vi "POST-Call.vi"(8 "error in (no error)":errorcluster, 9 "FunctionCall":T1, 10 "ApiKey":string, 11 "BaseUrl":string) -> (0 "error out":errorcluster, 3 "ToolReturn":cluster{"id":string, "result":variant})   [LabVIEW 2017]
uses:
  <vilib>/httpClient/POSTBuffer.vi
  <vilib>/httpClient/LabVIEWHTTPClient.lvlib
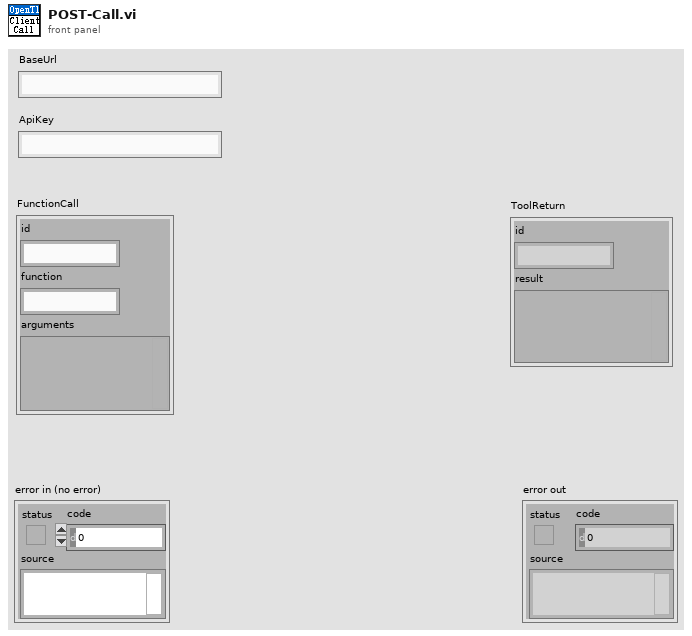
[diagram p1: front panel]
types:
  T1 = cluster{"id":string, "function":string, "arguments":variant}
  T2 = cluster{"jsonrpc":string, "id":string, "method":string, "params":variant}
  T3 = typedef "LabVIEWHTTPClient.lvlib/ClientHandle.ctl" = refnum<k1>
  T4 = cluster{"jsonrpc":string, "result":variant, "id":string, "JsonRPCHttpResponseBodyError":cluster{"code":i32, "message":string}}
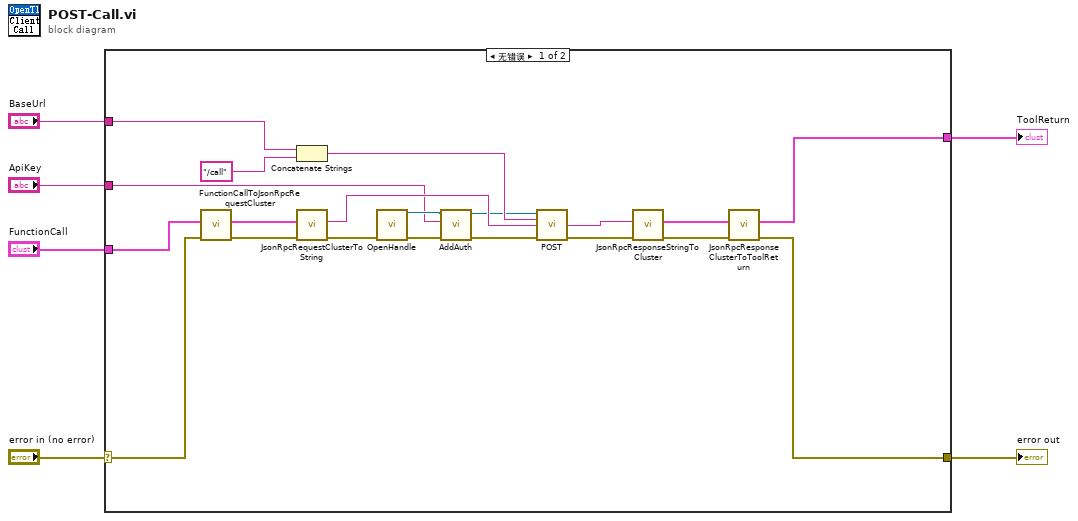
[diagram p0: block diagram]
diagram:
  n1 = case shown="无错误" "error in (no error)" {
    selector: "error in (no error)" -> [w16 w27]
    tunnel: [w17 w27] -> w5
    tunnel: "FunctionCall" -> [w26 _]
    tunnel: "BaseUrl" -> [w14 _]
    tunnel: [w18 _] -> w2
    tunnel: "ApiKey" -> [w7 _]
    frame No Error {
      n2 = call "FunctionCallToJsonRpcRequestCluster.vi"("error in (no error)"=w16, "FunctionCall"=w26) -> ("error out"=w24:errorcluster, "JsonRPCHttpRequestBody"=w25:T2)  [unwired: 8 in]
      n3 = Concatenate Strings(w14, "/call" ("字符串")) -> (w13:string)
      n4 = call "JsonRpcRequestClusterToString.vi"("error in (no error)"=w24, "JsonRPCHttpRequestBody"=w25) -> ("error out"=w12:errorcluster, "JsonRpcHttpRequestBodyJsonString"=w23:string)  [unwired: 8 in]
      n5 = call <vilib>:"OpenHandle.vi"("error in (no error)"=w12) -> ("client handle out"=w11:T3, "error out"=w9:errorcluster)  [unwired: 13 in]
      n6 = call "AddAuth.vi"("error in (no error)"=w9, "ApiKey"=w7, "client handle in"=w11) -> ("error out"=w8:errorcluster, "client handle out"=w10:T3)  [unwired: 7 in]
      n7 = call-poly <vilib>:"POST.vi"("client handle"=w10, "url"=w13, "buffer"=w23, "error in (no error)"=w8) -> ("body"=w22:string, "error out"=w21:errorcluster)  [unwired: 8 in, 2 out]
      n8 = call "JsonRpcResponseStringToCluster.vi"("error in (no error)"=w21, "JsonRpcResponseJsonString"=w22) -> ("error out"=w19:errorcluster, "JsonRPCHttpResponseBody"=w20:T4)  [unwired: 8 in]
      n9 = call "JsonRpcResponseClusterToToolReturn.vi"("error in (no error)"=w19, "JsonRPCHttpResponseBody"=w20) -> ("error out"=w17:errorcluster, "ToolReturn"=w18:cluster{"id":string, "result":variant})  [unwired: 8 in]
    }
    frame Error {
    }
  }
  "error out" <- w5
  "ToolReturn" <- w2
